vi "Add Project.vi"(7 "Project Store in":refnum<class "Project Store.lvclass">, 8 "error in (no error)":errorcluster, 11 "Name":string) -> (0 "error out":errorcluster, 3 "Project":T1, 5 "Project Store out":refnum<class "Project Store.lvclass">)   [LabVIEW 2024, in "Project Store.lvclass"]
doc: "Adds a new project to the in-memory model and returns its row. The project gets a new GUID as its ID, Active = TRUE, and Sort Order = the number of projects that existed before, so it sorts last. Nothing is written to disk - call Write to Data Source for that.\n\nGenerated by: Claude"
uses:
  Project Store.lvclass
  Rows/Project.ctl
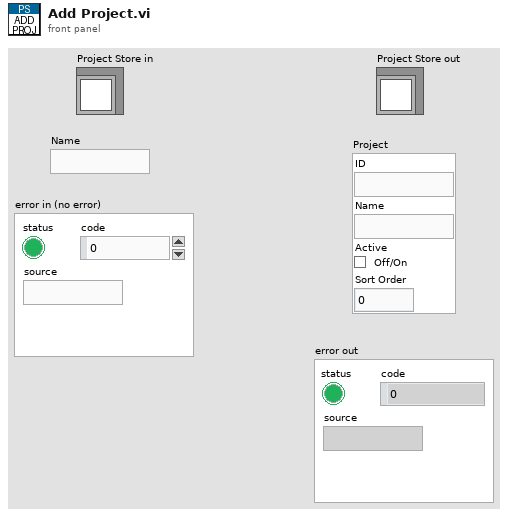
[diagram p1: front panel]
types:
  T1 = typedef "Project.ctl" = cluster{"ID":string, "Name":string, "Active":bool, "Sort Order":i32}
  T2 = typedef "Project List.ctl" = T1[]
  T3 = cluster{"NI GUID":string, "Name":string, "active":bool, i32}
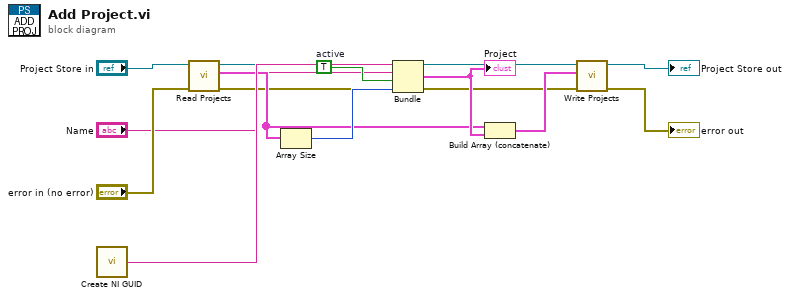
[diagram p0: block diagram]
diagram:
  w9 = TRUE  # active
  n1 = call <vilib>:"Create NI GUID.vi"() -> ("NI GUID"=w8:string)
  n2 = call-dynamic "Read Projects.vi"("error in (no error)"="error in (no error)", "Project Store in"="Project Store in") -> ("error out"=w4:errorcluster, "Project List"=w6:T2, "Project Store out"=w5:refnum<class "Project Store.lvclass">)  [unwired: 7 in]
  n3 = Array Size(array=w6) -> (size(s)=w7:i32)
  n4 = Bundle("NI GUID"=w8, "Name"="Name", "active"=w9, w7) -> (w10:T3)  [unwired: 1 in]
  "Project" <- w10
  n5 = Build Array (concatenate)(w6, w10) -> (w11:T2)
  n6 = call-dynamic "Write Projects.vi"("error in (no error)"=w4, "Project List"=w11, "Project Store in"=w5) -> ("error out"=→"error out":errorcluster, "Project Store out"=→"Project Store out":refnum<class "Project Store.lvclass">)  [unwired: 7 in]
